vi "set Marker Peak Search Type.vi"(8 "error in (no error)":errorcluster, 9 "Marker Index":i32, 10 "Peak Search Type":T1, 11 "Keysight 9020A in":refnum<class "Keysight 9020A.lvclass">) -> (0 "error out":errorcluster, 3 "Keysight 9020A out":refnum<class "Keysight 9020A.lvclass">)   [LabVIEW 2023, in "Spectrum Analyzer.lvlib" / "Keysight 9020A.lvclass"]
uses:
  Keysight 9020A.lvclass
  TYPE DEFINITION/TYPE Marker Peak Search Type.ctl
  Keysight 9020A.lvclass/Keysight 9020A.ctl
  Spectrum Analyzer.lvlib
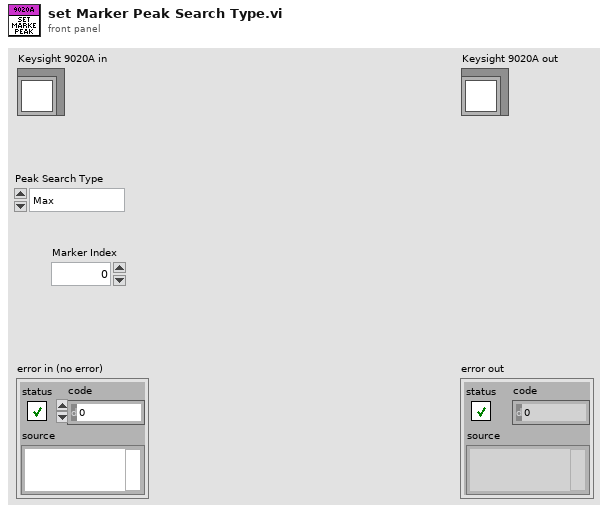
[diagram p1: front panel]
types:
  T1 = typedef "Spectrum Analyzer.lvlib/TYPE Marker Peak Search Type.ctl" = enum16{"Max", "Next Peak"}
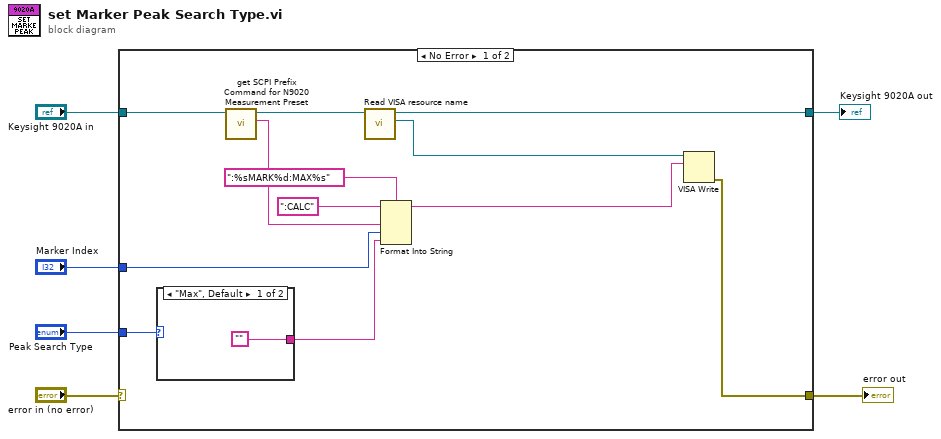
[diagram p0: block diagram]
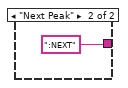
[diagram p2: hidden frame]
diagram:
  n1 = case shown="No Error" "error in (no error)" {
    selector: "error in (no error)" -> [_ w21]
    tunnel: "Keysight 9020A in" -> [w11 w22]
    tunnel: [w18 w22] -> w5
    tunnel: [w17 w21] -> w3
    tunnel: "Peak Search Type" -> [w16 _]
    tunnel: "Marker Index" -> [w9 _]
    frame No Error {
      n2 = case shown="\"Max\", Default" w16 {
        tunnel: ["" ":NEXT"] -> w8
        frame "Max", Default {
        }
        frame "Next Peak" {
        }
      }
      n3 = call "get SCPI Prefix Command for N9020 Measurement Preset.vi"("Keysight 9020A in"=w11) -> ("SCPI Prefix Command"=w12:string, "Keysight 9020A out"=w10:refnum<class "Keysight 9020A.lvclass">)  [unwired: 8 in, 1 out]
      n4 = call "Read VISA resource name.vi"("Keysight 9020A in"=w10) -> ("VISA resource name"=w15:refnum<visa-resource-name>, "Keysight 9020A out"=w18:refnum<class "Keysight 9020A.lvclass">)  [unwired: 8 in, 1 out]
      n5 = Format Into String(format string=":%sMARK%d:MAX%s", initial string=":CALC", w12, w9, w8) -> (resulting string=w7:string)  [unwired: 1 in, 1 out]
      n6 = VISA Write(VISA resource name=w15, write buffer=w7) -> (error out=w17:errorcluster)  [unwired: 1 in, 2 out]
    }
    frame Error {
    }
  }
  "error out" <- w3
  "Keysight 9020A out" <- w5
